vi "bitrate n2e.vi"(0 "number":u16 format="%0d", 1 "error in (no error)":errorcluster) -> (2 "error out":errorcluster, 3 "enum":T1)   [LabVIEW 2024, in "atsj peakcan basic.lvlib"]
uses:
  atsj peakcan basic.lvlib
  bitrate.ctl
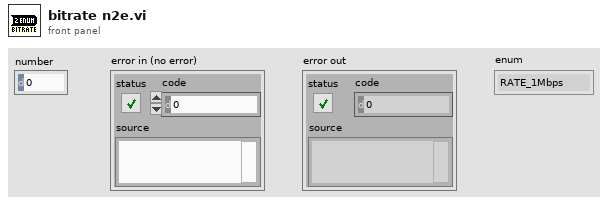
[diagram p1: front panel]
types:
  T1 = typedef "atsj peakcan basic.lvlib/bitrate.ctl" = enum16{"RATE_1Mbps", "RATE_800kbps", "RATE_500kbps", "RATE_250kbps", "RATE_125kbps", "RATE_100kbps", "RATE_95kbps", "RATE_83kbps", "RATE_50kbps", "RATE_47kbps", "RATE_33kbps", "RATE_20kbps", "RATE_10kbps", "RATE_5kbps"}
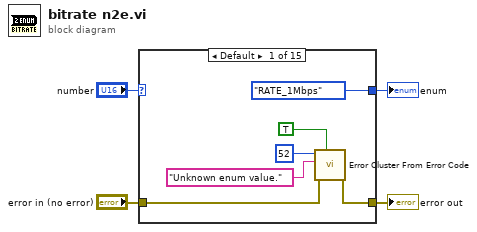
[diagram p0: block diagram]
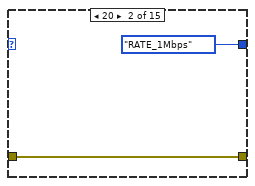
[diagram p2: hidden frame]
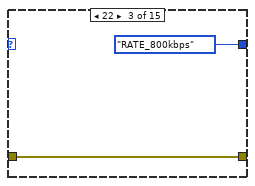
[diagram p3: hidden frame]
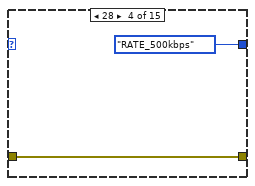
[diagram p4: hidden frame]
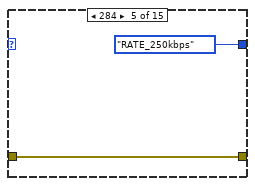
[diagram p5: hidden frame]
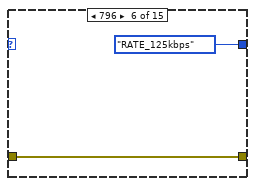
[diagram p6: hidden frame]
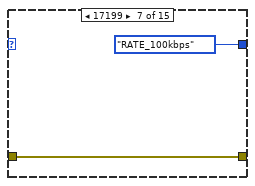
[diagram p7: hidden frame]
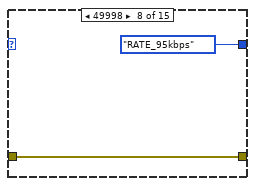
[diagram p8: hidden frame]
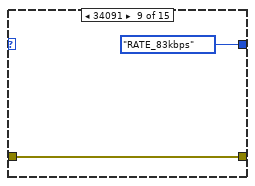
[diagram p9: hidden frame]
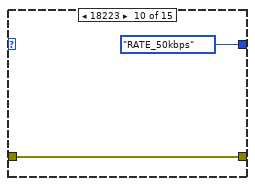
[diagram p10: hidden frame]
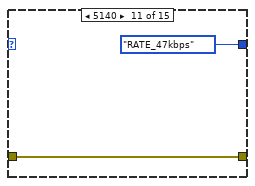
[diagram p11: hidden frame]
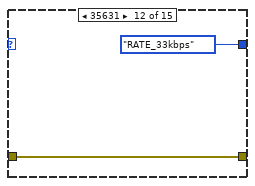
[diagram p12: hidden frame]
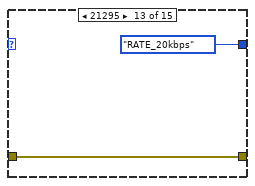
[diagram p13: hidden frame]
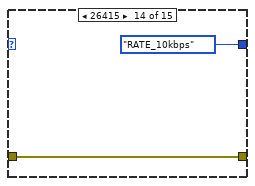
[diagram p14: hidden frame]
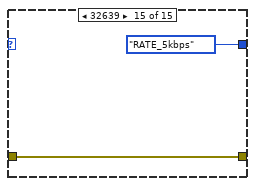
[diagram p15: hidden frame]
diagram:
  n1 = case shown="Default" "number" {
    tunnel: [bitrate."RATE_1Mbps" bitrate."RATE_1Mbps" bitrate."RATE_800kbps" bitrate."RATE_500kbps" bitrate."RATE_250kbps" bitrate."RATE_125kbps" bitrate."RATE_100kbps" bitrate."RATE_95kbps" bitrate."RATE_83kbps" bitrate."RATE_50kbps" bitrate."RATE_47kbps" bitrate."RATE_33kbps" bitrate."RATE_20kbps" bitrate."RATE_10kbps" bitrate."RATE_5kbps"] -> w3
    tunnel: [w8 w11 w13 w15 w17 w19 w21 w23 w25 w27 w29 w31 w33 w35 w37] -> w2
    tunnel: "error in (no error)" -> [w5 w11 w13 w15 w17 w19 w21 w23 w25 w27 w29 w31 w33 w35 w37]
    frame Default {
      n2 = call <vilib>:"Error Cluster From Error Code.vi"("show call chain? (False)"=TRUE, "error in (no error)"=w5, "error message (\"\")"="Unknown enum value.", "error code (0)"=52) -> ("error out"=w8:errorcluster)  [unwired: 5 in]
    }
    frame 20 {
    }
    frame 22 {
    }
    frame 28 {
    }
    frame 284 {
    }
    frame 796 {
    }
    frame 17199 {
    }
    frame 49998 {
    }
    frame 34091 {
    }
    frame 18223 {
    }
    frame 5140 {
    }
    frame 35631 {
    }
    frame 21295 {
    }
    frame 26415 {
    }
    frame 32639 {
    }
  }
  "enum" <- w3
  "error out" <- w2
